vi "set Marker State.vi"(7 "Marker Mode":T1, 8 "error in (no error)":errorcluster, 9 "trace index":i32, 10 "Marker Index":i32, 11 "Keysight 9020A in":refnum<class "Keysight 9020A.lvclass">) -> (0 "error out":errorcluster, 3 "Keysight 9020A out":refnum<class "Keysight 9020A.lvclass">)   [LabVIEW 2023, in "Spectrum Analyzer.lvlib" / "Keysight 9020A.lvclass"]
uses:
  Keysight 9020A.lvclass
  Keysight 9020A.lvclass/Keysight 9020A.ctl
  TYPE DEFINITION/TYPE Marker Control Mode.ctl
  Spectrum Analyzer.lvlib
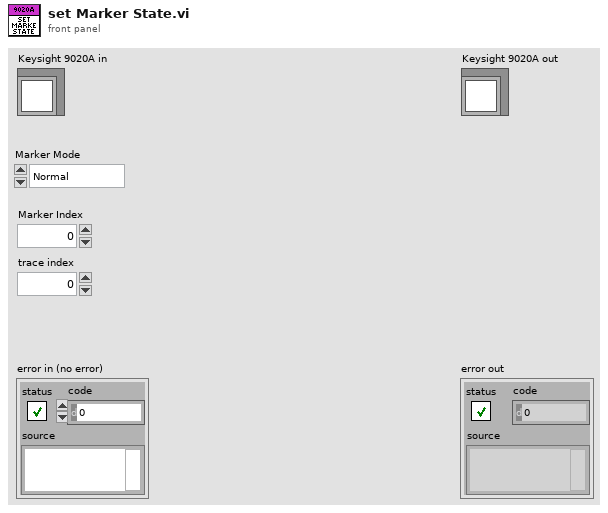
[diagram p1: front panel]
types:
  T1 = typedef "Spectrum Analyzer.lvlib/TYPE Marker Control Mode.ctl" = enum16{"Normal", "Delta", "Off"}
  T2 = typedef "Spectrum Analyzer.lvlib/TYPE Measurement Preset.ctl" = enum16{"Sweep SA Mode", "Channel Power", "Occupied BW", "ACP", "Spurious Emission", "Spurious Emission Mask", "Burst Power (Transmit Power)"}
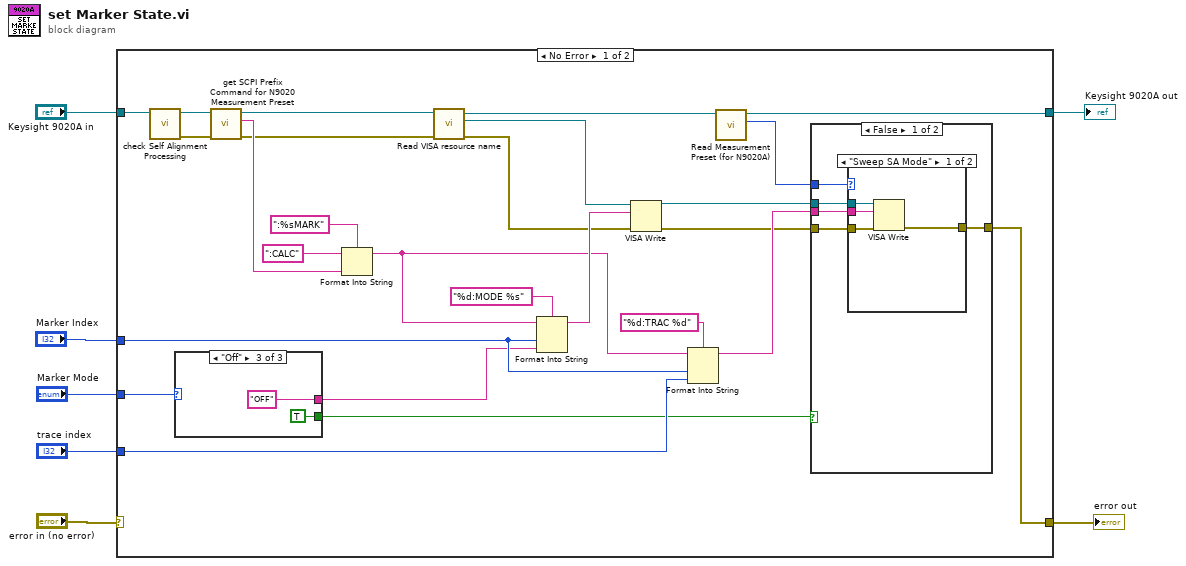
[diagram p0: block diagram]
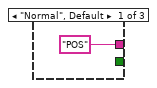
[diagram p4: hidden frame]
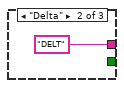
[diagram p5: hidden frame]
diagram:
  n1 = case shown="No Error" "error in (no error)" {
    selector: "error in (no error)" -> [_ w49]
    tunnel: "Keysight 9020A in" -> [w16 w50]
    tunnel: [w18 w50] -> w6
    tunnel: [w26 w49] -> w1
    tunnel: "Marker Index" -> [w29 _]
    tunnel: "trace index" -> [w11 _]
    tunnel: "Marker Mode" -> [w10 _]
    frame No Error {
      n2 = call "check Self Alignment Processing.vi"("Keysight 9020A in"=w16) -> ("error out"=w14:errorcluster, "Keysight 9020A out"=w15:refnum<class "Keysight 9020A.lvclass">)  [unwired: 8 in, 1 out]
      n3 = case shown="\"Off\"" w10 {
        tunnel: ["POS" "DELT" "OFF"] -> w9
        tunnel: [_ _ TRUE] -> w8
        frame "Normal", Default {
        }
        frame "Delta" {
        }
        frame "Off" {
        }
      }
      n4 = call "get SCPI Prefix Command for N9020 Measurement Preset.vi"("error in (no error)"=w14, "Keysight 9020A in"=w15) -> ("error out"=w13:errorcluster, "SCPI Prefix Command"=w22:string, "Keysight 9020A out"=w21:refnum<class "Keysight 9020A.lvclass">)  [unwired: 7 in]
      n5 = Format Into String(format string=":%sMARK", initial string=":CALC", w22) -> (resulting string=w20:string)  [unwired: 1 in, 1 out]
      n6 = call "Read VISA resource name.vi"("error in (no error)"=w13, "Keysight 9020A in"=w21) -> ("error out"=w12:errorcluster, "VISA resource name"=w25:refnum<visa-resource-name>, "Keysight 9020A out"=w19:refnum<class "Keysight 9020A.lvclass">)  [unwired: 7 in]
      n7 = Format Into String(format string="%d:MODE %s", initial string=w20, w29, w9) -> (resulting string=w33:string)  [unwired: 1 in, 1 out]
      n8 = VISA Write(VISA resource name=w25, write buffer=w33, error in (no error)=w12) -> (VISA resource name out=w31:refnum<visa-resource-name>, error out=w27:errorcluster)  [unwired: 1 out]
      n9 = Format Into String(format string="%d:TRAC %d", initial string=w20, w29, w11) -> (resulting string=w28:string)  [unwired: 1 in, 1 out]
      n10 = call "Read Measurement Preset (for N9020A).vi"("Keysight 9020A in"=w19) -> ("Measurement Preset"=w17:T2, "Keysight 9020A out"=w18:refnum<class "Keysight 9020A.lvclass">)  [unwired: 8 in, 1 out]
      n11 = case shown="False" w8 {
        tunnel: w31 -> [w38 _]
        tunnel: w28 -> [w37 _]
        tunnel: w27 -> [w36 w44]
        tunnel: [w35 w44] -> w26
        tunnel: w17 -> [w34 _]
        frame False {
          n12 = case shown="\"Sweep SA Mode\"" w34 {
            tunnel: w38 -> [w42 _]
            tunnel: w37 -> [w41 _]
            tunnel: w36 -> [w40 w43]
            tunnel: [w39 w43] -> w35
            frame "Sweep SA Mode" {
              n13 = VISA Write(VISA resource name=w42, write buffer=w41, error in (no error)=w40) -> (error out=w39:errorcluster)  [unwired: 2 out]
            }
            frame Default {
            }
          }
        }
        frame True {
        }
      }
    }
    frame Error {
    }
  }
  "error out" <- w1
  "Keysight 9020A out" <- w6
